vi "virtuino_labview.vi"() -> ()   [LabVIEW 2024]
panel:
  in  "Dial":dbl(knob) scale=0.0..100.0
  in  "Boolean":bool
  out "led":bool
  out "Thermometer":dbl(slide) scale=0.0..100.0
  out "data out":string
  in  "remote port or service name":u16=200
  in  "address":string="192.168.4.1"
  in  "stop":bool
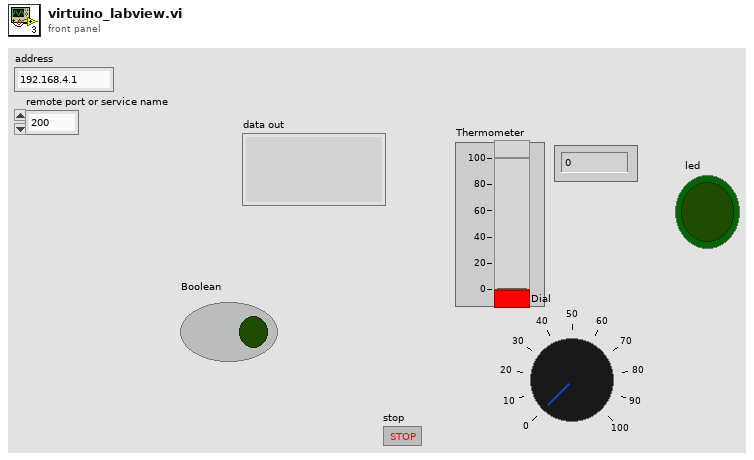
[diagram p1: front panel]
types:
  T1 = enum16{"Standard", "Buffered", "CRLF", "Immediate"}
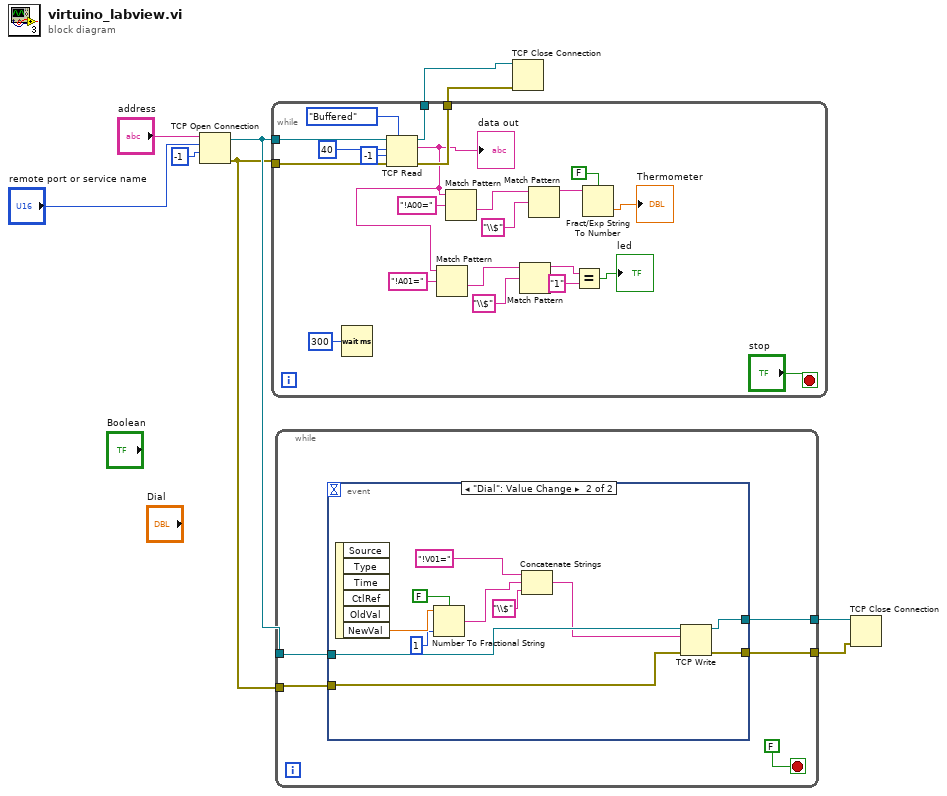
[diagram p0: block diagram]
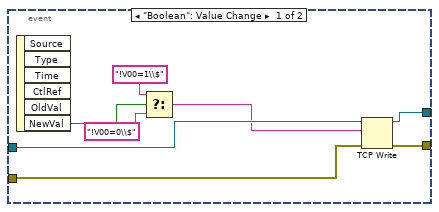
[diagram p2: hidden frame]
diagram:
  n1 = TCP Open Connection(address="address", remote port or service name="remote port or service name", timeout ms (60000)=-1) -> (connection ID=w4:refnum<k5>, error out=w3:errorcluster)  [unwired: 2 in]
  n2 = while {
    tunnel: w4 -> [w30]
    tunnel: w3 -> [w29]
    tunnel: [w25] -> w6
    tunnel: [w24] -> w5
    stop <- "stop" stop-if-true
    n3 = Wait (ms)(milliseconds to wait=u32 300) -> ()  [unwired: 1 out]
    n4 = TCP Read(connection ID=w30, bytes to read=40, error in (no error)=w29, 7:T1."Buffered" ("mode (standard)"), 9:-1 ("timeout ms (25000)")) -> (connection ID out=w24:refnum<k5>, data out=w13:string, error out=w25:errorcluster)
    "data out" <- w13
    n5 = Match Pattern(string=w13, regular expression="!A01=") -> (after substring=w15:string)  [unwired: 1 in, 3 out]
    n6 = Match Pattern(string=w13, regular expression="!A00=") -> (after substring=w21:string)  [unwired: 1 in, 3 out]
    n7 = Match Pattern(string=w15, regular expression="\\$") -> (before substring=w12:string)  [unwired: 1 in, 3 out]
    n8 = Match Pattern(string=w21, regular expression="\\$") -> (before substring=w19:string)  [unwired: 1 in, 3 out]
    n9 = Equal?(x=w12, y="1") -> (x = y?=→"led":bool)
    n10 = Fract/Exp String To Number(use system decimal point (T)=FALSE, string=w19) -> (number=→"Thermometer":dbl)  [unwired: 2 in, 1 out]
  }
  n11 = while {
    tunnel: w4 -> [w35]
    tunnel: w3 -> [w34]
    tunnel: [w33] -> w2
    tunnel: [w32] -> w1
    stop <- FALSE stop-if-true
    n12 = event shown="[1] \"Dial\": Value Change" {
      selector: _ -> [_ _]
      dyn-events: _ -> [_ _]
      timeout: _ -> [_ _]
      tunnel: w35 -> [w44 w55]
      tunnel: w34 -> [w43 w54]
      tunnel: [w42 w53] -> w33
      tunnel: [w41 w52] -> w32
      event "Boolean": Value Change {
        n13 = event-data() -> ("NewVal"=w40:bool)  [unwired: 1 in, 5 out]
        n14 = Select(t="!V00=1\\$", s=w40, f="!V00=0\\$") -> (s? t:f=w37:string)
        n15 = TCP Write(connection ID=w44, data in=w37, error in (no error)=w43) -> (connection ID out=w42:refnum<k5>, error out=w41:errorcluster)  [unwired: 1 in, 1 out]
      }
      event "Dial": Value Change {
        n16 = event-data() -> ("NewVal"=w49:dbl)  [unwired: 1 in, 5 out]
        n17 = Number To Fractional String(use system decimal point (T)=FALSE, number=w49, precision (6)=i16 1) -> (F-format string=w46:string)  [unwired: 1 in]
        n18 = Concatenate Strings("!V01=", w46, "\\$" ("string")) -> (w45:string)
        n19 = TCP Write(connection ID=w55, data in=w45, error in (no error)=w54) -> (connection ID out=w53:refnum<k5>, error out=w52:errorcluster)  [unwired: 1 in, 1 out]
      }
    }
  }
  n20 = TCP Close Connection(connection ID=w5, error in (no error)=w6) -> ()  [unwired: 1 in, 2 out]
  n21 = TCP Close Connection(connection ID=w2, error in (no error)=w1) -> ()  [unwired: 1 in, 2 out]
